vi "Disk_Usage.vi"() -> (3 "usage %":dbl)   [LabVIEW 2025]
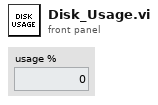
[diagram p1: front panel]
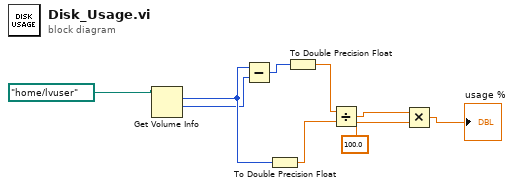
[diagram p0: block diagram]
diagram:
  n1 = Get Volume Info(11:path "/home/lvuser" ("path")) -> (1:w2:i64, 2:w7:i64)  [unwired: 1 in, 4 out]
  n2 = Subtract(x=w7, y=w2) -> (x-y=w5:i64)
  n3 = To Double Precision Float(number=w7) -> (double precision float=w8:dbl)
  n4 = To Double Precision Float(number=w5) -> (double precision float=w6:dbl)
  n5 = Divide(x=w6, y=w8) -> (x/y=w3:dbl)
  n6 = Multiply(x=w3, y=100.0) -> (x*y=→"usage %":dbl)
